vi "Launch User Control Module Scripting Utility.vi"   [LabVIEW 2014]
uses:
  control module/script/FromClusterToTagBusScript.vi
  control module/script/control module data interface generator.lvlib
types:
  T1 = enum32{"Invalid", "Standard", "Closed", "Hidden", "Minimized", "Maximized"}
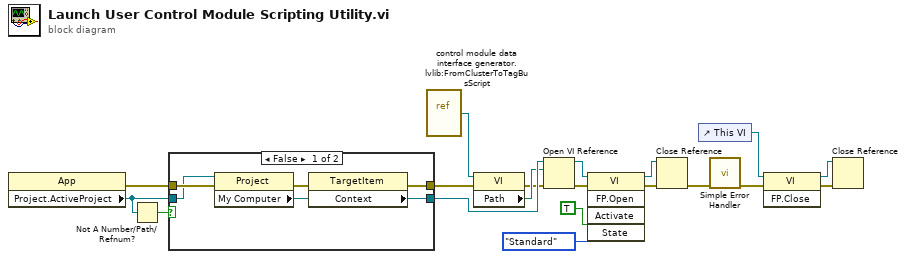
[diagram p0: block diagram]
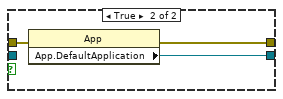
[diagram p2: hidden frame]
diagram:
  n1 = property class="App"() -> (error out=w18:errorcluster, "Project.ActiveProject"=w7:refnum<vi>)  [unwired: 2 in, 1 out]
  n2 = Not A Number/Path/Refnum?(number/path/refnum=w7) -> (NaN/Path/Refnum?=w6:bool)
  n3 = case shown="False" w6 {
    tunnel: w18 -> [w25 w28]
    tunnel: [w20 w26] -> w17
    tunnel: [w22 w27] -> w14
    tunnel: w7 -> [w23 _]
    frame False {
      n4 = property class="Project"(reference=w23, error in=w25) -> (error out=w24:errorcluster, "My Computer"=w21:refnum<vi>)  [unwired: 1 out]
      n5 = property class="TargetItem"(reference=w21, error in=w24) -> (error out=w22:errorcluster, "Context"=w20:refnum<vi>)  [unwired: 1 out]
    }
    frame True {
      n6 = property class="App"(error in=w28) -> (error out=w27:errorcluster, "App.DefaultApplication"=w26:refnum<vi>)  [unwired: 1 in, 1 out]
    }
  }
  n7 = vi-ref "control module data interface generator.lvlib:FromClusterToTagBusScript.vi"() -> (w19:refnum<vi>)
  n8 = property class="VI"(reference=w19, error in=w14) -> (error out=w15:errorcluster, "Path"=w16:path)  [unwired: 1 out]
  n9 = Open VI Reference(application reference (local)=w17, vi path=w16, error in (no error)=w15) -> (vi reference=w12:refnum<vi>, error out=w13:errorcluster)  [unwired: 3 in]
  n10 = invoke class="VI" method="FP.Open"(reference=w12, error in=w13, "Activate"=TRUE ("Activate?"), "State"=T1."Standard") -> (reference out=w10:refnum<vi>, error out=w11:errorcluster)  [unwired: 1 in, 3 out]
  n11 = Close Reference(reference=w10, error in (no error)=w11) -> (error out=w5:errorcluster)
  n12 = control-ref of="This VI"() -> (w3:refnum<vi>)
  n13 = call <vilib>:"Simple Error Handler.vi"("error in (no error)"=w5) -> ("error out"=w4:errorcluster)  [unwired: 4 in, 4 out]
  n14 = invoke class="VI" method="FP.Close"(reference=w3, error in=w4) -> (reference out=w1:refnum<vi>, error out=w2:errorcluster)  [unwired: 1 in, 1 out]
  n15 = Close Reference(reference=w1, error in (no error)=w2) -> ()  [unwired: 1 out]
